vi "Create Frame Buffer.vi"(8 "error in":errorcluster, 11 "GUID":string) -> (0 "error out":errorcluster)   [LabVIEW 2025, in "CAN-LIN Raw Bus Capture.lvclass"]
uses:
  CAN-LIN Raw Bus Capture.lvclass
  CAN-LIN Raw Bus Capture.lvclass/CAN-LIN Raw Bus Capture.ctl
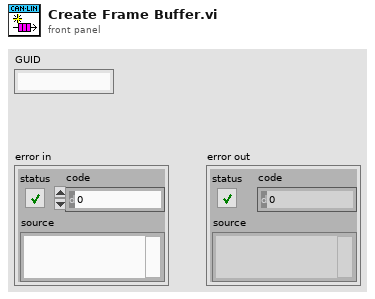
[diagram p1: front panel]
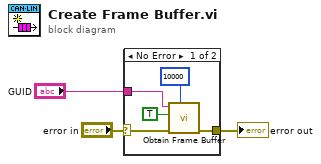
[diagram p0: block diagram]
diagram:
  n1 = case shown="No Error" "error in" {
    selector: "error in" -> [w7 w9]
    tunnel: [w8 w9] -> w2
    tunnel: "GUID" -> [w4 _]
    frame No Error {
      n2 = call "Obtain Frame Buffer.vi"("Buffer Size (10k)"=10000, "error in"=w7, "Create (F)"=TRUE ("create if not found? (T)"), "GUID"=w4) -> ("error out"=w8:errorcluster)  [unwired: 6 in, 1 out]
    }
    frame Error {
    }
  }
  "error out" <- w2
